vi "create.from_array.vi"(8 "error in":errorcluster, 10 "labels":string[](array[string])) -> (0 "error out":errorcluster, 3 "labels out":refnum<class "labels.lvclass">)   [LabVIEW 2020, in "nominal types.lvlib" / "labels.lvclass"]
uses:
  labels.lvclass
  labels.lvclass/labels.ctl
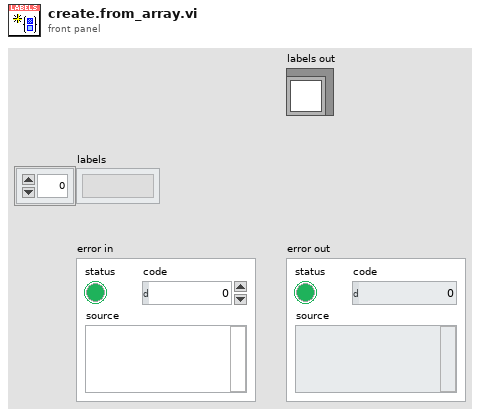
[diagram p1: front panel]
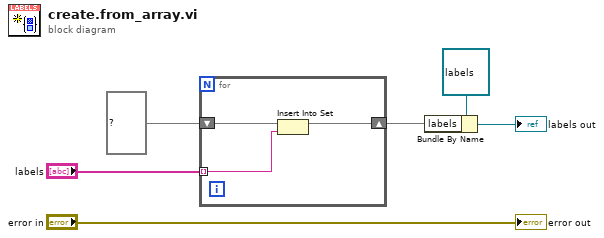
[diagram p0: block diagram]
diagram:
  n1 = for {
    shift-right: [w8] -> w4
    shift-left: set{string} {} ("labels") -> [w9]
    tunnel: "labels" -> [w7] mode=indexing
    n2 = Insert Into Set(10:w7, 11:w9) -> (3:w8:set{string})  [unwired: 1 out]
  }
  n3 = Bundle By Name(cluster=refnum<class "labels.lvclass"> refnum ("properties out"), "labels"=w4) -> (→"labels out":refnum<class "labels.lvclass">)
  "error out" <- "error in"
